vi "Apply Setpoints.vi"(8 "error in":errorcluster, 10 "setpoints":T1[](array[typedef]), 11 "VTU Sim Rig in":refnum<class "VTU Sim Rig.lvclass">) -> (0 "error out":errorcluster, 3 "VTU Sim Rig out":refnum<class "VTU Sim Rig.lvclass">)   [LabVIEW 2026, in "VTU Sim Rig.lvclass"]
doc: "VTU Sim Rig override of Rig:Apply Setpoints. Stores the commanded setpoints; the simulation moves its state toward them on each Tick."
uses:
  VTU Sim Rig.lvclass
  VTU Sim Rig.lvclass/VTU Sim Rig.ctl
  src/Typedefs/Channel Value.ctl
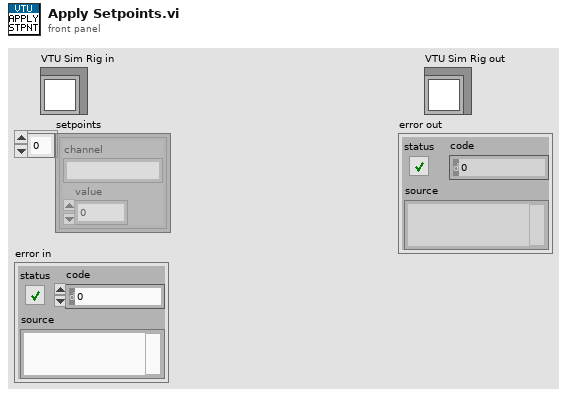
[diagram p1: front panel]
types:
  T1 = typedef "Channel Value.ctl" = cluster{"channel":string, "value":dbl}
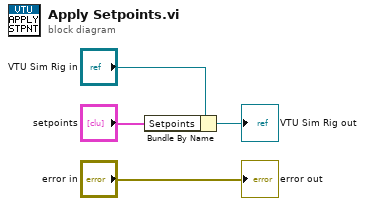
[diagram p0: block diagram]
diagram:
  n1 = Bundle By Name(cluster="VTU Sim Rig in", "Setpoints"="setpoints") -> (→"VTU Sim Rig out":refnum<class "VTU Sim Rig.lvclass">)
  "error out" <- "error in"
